vi "for loop.vi"() -> ()   [LabVIEW 2018]
panel:
  out "Numeric":dbl
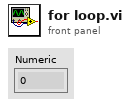
[diagram p1: front panel]
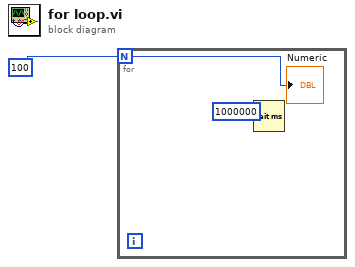
[diagram p0: block diagram]
diagram:
  n1 = for {
    N: 100 -> [w2]
    n2 = Wait (ms)(milliseconds to wait=1000000) -> ()  [unwired: 1 out]
    "Numeric" <- w2
  }
